vi "Own20261012_SelectProperties.vi"() -> ()   [LabVIEW 2024]
panel:
  out "property_item_ids":refnum<vi>[](array[refnum])
  in  "property_id_strings":string[](array[string])
  in  "allow_alternate_names":bool
  out "error out":errorcluster caption="错误输出"
  in  "property_id":u32
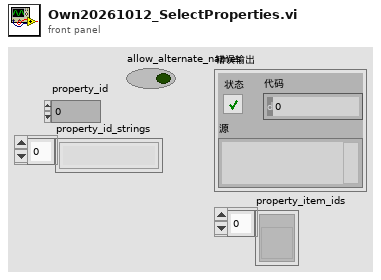
[diagram p1: front panel]
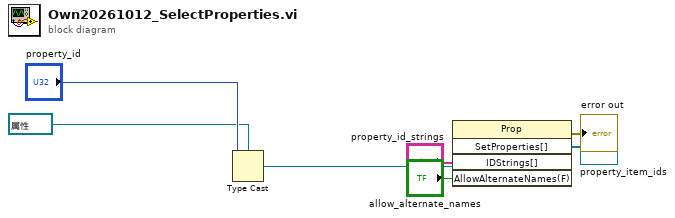
[diagram p0: block diagram]
diagram:
  n1 = Type Cast(type=refnum<vi> refnum ("引用"), x="property_id") -> (*(type *) &x=w5:refnum<vi>)
  n2 = invoke class="Prop" method="SetProperties[]"(reference=w5, "IDStrings[]"="property_id_strings", "AllowAlternateNames(F)"="allow_alternate_names") -> (error out=→"error out":errorcluster, "SetProperties[]"=→"property_item_ids":refnum<vi>[])  [unwired: 2 in, 3 out]
